vi "while loop.vi"() -> ()   [LabVIEW 2021]
panel:
  out "Numeric 4":i32
  out "Numeric 3":dbl
  in  "Numeric 2":dbl
  in  "Numeric":dbl
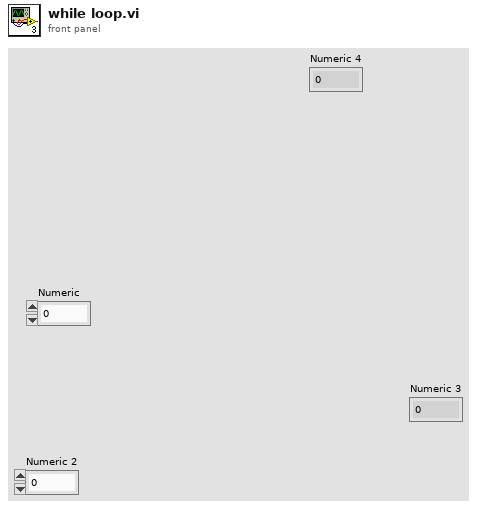
[diagram p1: front panel]
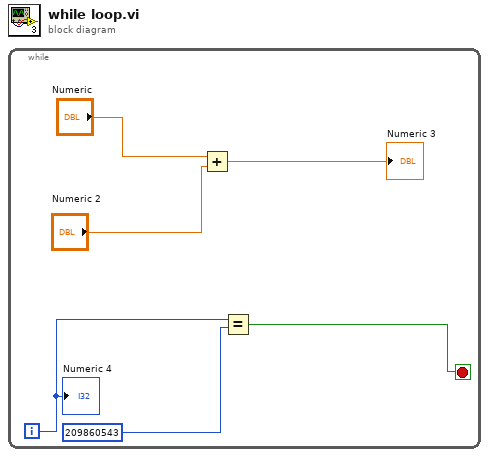
[diagram p0: block diagram]
diagram:
  n1 = while {
    i -> [w3]
    stop <- w2 stop-if-true
    n2 = Add(x="Numeric", y="Numeric 2") -> (x+y=→"Numeric 3":dbl)
    n3 = Equal?(x=w3, y=209860543) -> (x = y?=w2:bool)
    "Numeric 4" <- w3
  }
